vi "SPARK Get Closed Loop Config.vi"   [LabVIEW 2027]
doc: "Get the configuration of the closed loop controller of the SPARK."
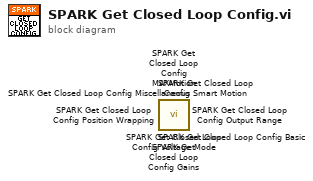
[diagram p0: block diagram]
diagram:
  n1 = call <vilib>:"SPARK Get Closed Loop Config Voltage Mode.vi"() -> ()  [unwired: 9 in, 3 out]
  n2 = call <vilib>:"SPARK Get Closed Loop Config Smart Motion.vi"() -> ()  [unwired: 6 in, 6 out]
  n3 = call <vilib>:"SPARK Get Closed Loop Config Position Wrapping.vi"() -> ()  [unwired: 7 in, 5 out]
  n4 = call <vilib>:"SPARK Get Closed Loop Config Output Range.vi"() -> ()  [unwired: 8 in, 4 out]
  n5 = call <vilib>:"SPARK Get Closed Loop Config Miscellaneous.vi"() -> ()  [unwired: 7 in, 5 out]
  n6 = call <vilib>:"SPARK Get Closed Loop Config MAXMotion.vi"() -> ()  [unwired: 7 in, 5 out]
  n7 = call <vilib>:"SPARK Get Closed Loop Config Gains.vi"() -> ()  [unwired: 7 in, 5 out]
  n8 = call <vilib>:"SPARK Get Closed Loop Config Basic.vi"() -> ()  [unwired: 8 in, 4 out]
